vi "Main_Rover_Control.vi"() -> ()   [LabVIEW 2022 SP3]
doc: "Rows start at (0,0). Positive field inputs. Run once, Send Path, wait Path ready, Start. Persistent command replies exclude heartbeat. No headland."
panel:
  in  "Seed spacing cm (10 or 20)":i32=10
  in  "Enable planting":bool=TRUE
  out "Graph layout error":errorcluster
  in  "Orientation":enum16{"Run Along Length", "Run Along Width"}(ring)
  out "XY Graph":cluster{dbl[], dbl[]}(graph)={[0.0, 0.0, 2.0, 2.0, 4.0, 4.0, 6.0, 6.0], [0.0, 8.0, 8.0, 0.0, 0.0, 8.0, 8.0, 0.0]}
  in  "Row Spacing":dbl=2.0
  in  "Field Length":dbl=8.0
  in  "Field Width":dbl=6.0
  out "Field inputs valid":bool
  out "Connection error":errorcluster
  out "Expected acknowledgement":string
  out "Run status":string="Stopped"
  out "Last rover error":string
  out "Connected":bool
  out "Calibration valid":bool
  out "Running estimate":bool
  out "Path ready":bool
  out "Current command":string
  out "Last received line":string
  in  "Disconnect":bool
  in  "Reset E-stop":bool
  in  "E-STOP":bool
  in  "STOP":bool
  in  "Start":bool
  in  "Send Path":bool
  out "Path points":i32
  out "Greeting":string
  in  "Initial heading degrees":dbl=90.0
  in  "Right 90 ms - calibrate":dbl=925.0
  in  "Left 90 ms - calibrate":dbl=925.0
  in  "Forward ms per cm":dbl=40.0
  in  "TCP port":u16=5000
  in  "ESP32 address":string="192.168.4.1"
  # "ROVER PATH CONTROL"
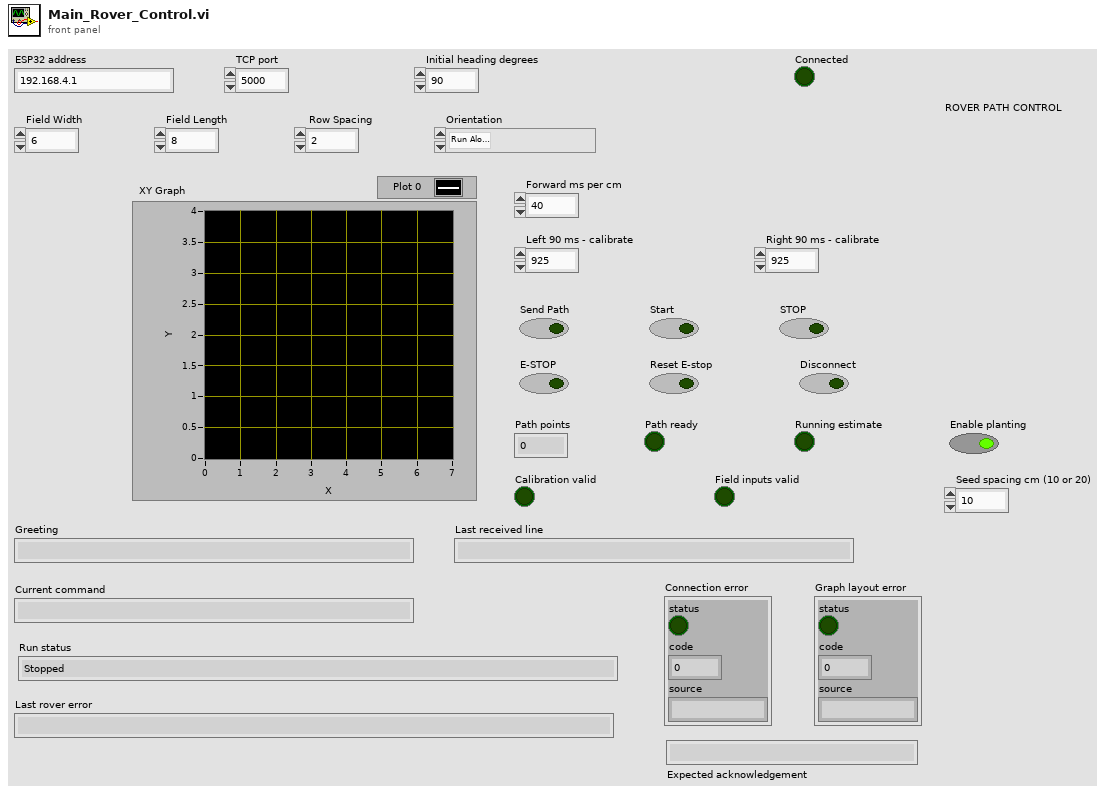
[diagram p1: front panel]
diagram:
  w97 = cluster{"Width":u32, "Height":u32} {"Width"=250, "Height"=250}  # Plot size
  w92 = 2.0  # x
  w88 = 3.0  # Safe s
  w86 = 6.0  # Safe l
  w84 = 5.0  # Safe w
  w83 = errorcluster {"status"=FALSE, "code"=0, "source"=""}  # Input error template
  w76 = 100  # Final timeout
  w75 = "STOP\r\n"  # Final STOP
  w70 = ""  # lastline initial
  w69 = ""  # wanted initial
  w68 = ""  # buffer initial
  w67 = 0  # oldreset initial
  w66 = 0  # oldestop initial
  w65 = 0  # oldstop initial
  w64 = 0  # oldstart initial
  w63 = 0  # oldsend initial
  w62 = 0  # lastreceive initial
  w61 = 0  # lastping initial
  w60 = 0  # running initial
  w59 = 0  # ready initial
  w58 = 0  # deadline initial
  w57 = 0  # pending initial
  w56 = -1  # position initial
  w51 = "HELLO,ROVER,2,CM_PER_UNIT=10\r\n"  # Expected greeting
  w47 = 30  # Greeting bytes
  w44 = 3000  # Connect timeout
  w41 = 3  # Decimals
  w40 = "START,"  # Start prefix
  w30 = "OK,CAL"  # Calibration acknowledgement
  w26 = 3  # Decimals
  w25 = ","  # Comma
  w23 = 3  # Decimals
  w22 = ","  # Comma
  w20 = 3  # Decimals
  w19 = "CAL,"  # CAL
  n1 = property on="XY Graph" class="XYGraph (strict)"("Plot Area:Size"=w97) -> (error out=→"Graph layout error":errorcluster)  [unwired: 2 in, 1 out]
  n2 = Number To Fractional String(number="Forward ms per cm", precision (6)=w20) -> (F-format string=w21:string)  [unwired: 2 out]
  n3 = Number To Fractional String(number="Left 90 ms - calibrate", precision (6)=w23) -> (F-format string=w24:string)  [unwired: 2 out]
  n4 = Number To Fractional String(number="Right 90 ms - calibrate", precision (6)=w26) -> (F-format string=w27:string)  [unwired: 2 out]
  n5 = Build Array(w30) -> (w31:string[])
  n6 = Number To Fractional String(number="Initial heading degrees", precision (6)=w41) -> (F-format string=w42:string)  [unwired: 2 out]
  n7 = TCP Open Connection(address="ESP32 address", remote port or service name="TCP port", timeout ms (60000)=w44) -> (connection ID=w45:refnum<k5>, error out=w46:errorcluster)  [unwired: 2 in]
  n8 = To Long Integer(number="Orientation") -> (32bit integer=w80:i32)
  n9 = Select(t="PLANT,1,", s="Enable planting", f="PLANT,0,") -> (s? t:f=w102:string)
  n10 = Number To Decimal String(number="Seed spacing cm (10 or 20)") -> (decimal integer string=w103:string)  [unwired: 1 in]
  n11 = Build Array("OK,PLANT") -> (w35:string[])
  n12 = Concatenate Strings(w19, w21, w22, w24, w25, w27) -> (w28:string)
  n13 = Concatenate Strings(w40, w42) -> (w43:string)
  n14 = TCP Read(connection ID=w45, bytes to read=w47, error in (no error)=w46, 9:w44) -> (connection ID out=w48:refnum<k5>, data out=w49:string, error out=w50:errorcluster)  [unwired: 1 in]
  "Greeting" <- w49
  "Connection error" <- w50
  n15 = formula code="int32 ok;float64 cross;ok=(w>0 && w<=1000 && l>0 && l<=1000 && s>0 && s<=1000 && (o==0 || o==1));if(ok){cross=w;if(o==1){cross=l;}ok=(cross/s<=127);}"("w"="Field Width", "l"="Field Length", "s"="Row Spacing", "o"=w80) -> ("ok"=w78:i32)
  n16 = Concatenate Strings(w102, w103) -> (w104:string)
  n17 = Build Array(w28) -> (w29:string[])
  n18 = Equal?(x=w49, y=w51) -> (x = y?=w52:bool)
  n19 = Unbundle By Name(w50) -> ("status"=w55:bool)
  n20 = Not Equal To 0?(x=w78) -> (x != 0?=w81:bool)
  "Field inputs valid" <- w81
  n21 = Build Array(w104) -> (w33:string[])
  n22 = Not(x=w81) -> (.not. x?=w82:bool)
  n23 = Select(t="Field Width", s=w81, f=w84) -> (s? t:f=w85:dbl)
  n24 = Select(t="Field Length", s=w81, f=w86) -> (s? t:f=w87:dbl)
  n25 = Select(t="Row Spacing", s=w81, f=w88) -> (s? t:f=w89:dbl)
  n26 = Bundle By Name(cluster=w83, "status"=w82) -> (w54:errorcluster)
  n27 = call "Generate_Rows.vi"("Orientation"="Orientation", "Row Spacing"=w89, "Field Length"=w87, "Field Width"=w85) -> ("Waypoints"=w93:cluster{"X":dbl, "Y":dbl, "Seed":bool}[][])  [unwired: 11 in]
  n28 = Unbundle By Name(w54) -> ("status"=w53:bool)
  n29 = Array Size(array=w93) -> (size(s)=w94:i32[])
  n30 = Index Array(array=w94) -> (element=w95:i32)  [unwired: 1 in]
  n31 = Multiply(x=w92, y=w95) -> (x*y=w96:dbl)
  n32 = for {
    N: w96 -> [_]
    tunnel: w93 -> [w111]
    tunnel: [w113] -> w11 mode=indexing
    tunnel: [w112] -> w10 mode=indexing
    tunnel: [w114] -> w12 mode=indexing
    i -> [w106]
    w107 = 2  # y
    n33 = Quotient & Remainder(x=w106, y=w107) -> (x-y*floor(x/y)=w109:i32, floor(x/y)=w108:i32)
    n34 = Index Array(array=w111, index (row)=w108, index (col)=w109) -> (element=w110:cluster{"X":dbl, "Y":dbl, "Seed":bool})
    n35 = Unbundle By Name(w110) -> ("X"=w112:dbl, "Y"=w113:dbl, "Seed"=w114:bool)
  }
  n36 = call "Rover_Planting_Commands.vi"("X"=w10, "Y"=w11, "Seeds"=w12) -> ("Commands"=w7:string[], "Expected"=w8:string[], "Count"=w9:i32)  [unwired: 10 in]
  "Path points" <- w9
  n37 = Array Size(array=w11) -> (size(s)=w13:i32)
  n38 = Bundle(w10, w11) -> (→"XY Graph":cluster{dbl[], dbl[]})  [unwired: 1 in]
  n39 = formula code="int32 ok,i;ok=(n>=2 && n<=256 && n==ny);if(ok){for(i=0;i<n;i++){if(!(x[i]>=-0.000001 && x[i]<=w+0.000001 && y[i]>=-0.000001 && y[i]<=l+0.000001)){ok=0;}}}"("n"=w9, "ny"=w13, "x"=w10, "y"=w11, "w"="Field Width", "l"="Field Length") -> ("ok"=w14:i32)
  n40 = formula code="int32 valid; valid=((spacing==10 || spacing==20) && n>=2 && n<=256 && n==ny && ms>=1 && ms<=1000 && l>=1 && l<=10000 && r>=1 && r<=10000 && h>=-180 && h<=180);"("n"=w9, "ny"=w13, "ms"="Forward ms per cm", "l"="Left 90 ms - calibrate", "r"="Right 90 ms - calibrate", "h"="Initial heading degrees", "spacing"="Seed spacing cm (10 or 20)") -> ("valid"=w17:i32)
  n41 = Build Array (concatenate)(w29, w7, w33) -> (w32:string[])
  n42 = Build Array (concatenate)(w31, w8, w35) -> (w34:string[])
  n43 = Not Equal To 0?(x=w17) -> (x != 0?=w36:bool)
  n44 = Select(t=w32, s=w36, f=w7) -> (s? t:f=w37:string[])
  n45 = Select(t=w34, s=w36, f=w8) -> (s? t:f=w38:string[])
  n46 = Array Size(array=w37) -> (size(s)=w39:i32)
  n47 = while {
    shift-right: [w129] -> _
    shift-left: w56 -> [w128]
    shift-right: [w131] -> _
    shift-left: w57 -> [w130]
    shift-right: [w133] -> _
    shift-left: w58 -> [w132]
    shift-right: [w135] -> _
    shift-left: w59 -> [w134]
    shift-right: [w137] -> _
    shift-left: w60 -> [w136]
    shift-right: [w139] -> _
    shift-left: w61 -> [w138]
    shift-right: [w141] -> _
    shift-left: w62 -> [w140]
    shift-right: [w143] -> _
    shift-left: w63 -> [w142]
    shift-right: [w145] -> _
    shift-left: w64 -> [w144]
    shift-right: [w147] -> _
    shift-left: w65 -> [w146]
    shift-right: [w149] -> _
    shift-left: w66 -> [w148]
    shift-right: [w151] -> _
    shift-left: w67 -> [w150]
    shift-right: [w153] -> _
    shift-left: w68 -> [w152]
    shift-right: [w155] -> _
    shift-left: w69 -> [w154]
    shift-right: [w229] -> _
    shift-left: w70 -> [w228]
    shift-right: [w232] -> _
    shift-left: "" -> [w239]
    shift-right: [w244] -> _
    shift-left: "" -> [w243]
    shift-right: [w246] -> _
    shift-left: 0 -> [w201]
    tunnel: w48 -> [w116]
    tunnel: w43 -> [w122]
    tunnel: w52 -> [w123]
    tunnel: w55 -> [w124]
    tunnel: w53 -> [w125]
    tunnel: w17 -> [w120]
    tunnel: w14 -> [w121]
    tunnel: w37 -> [w117]
    tunnel: w38 -> [w118]
    tunnel: w39 -> [w119]
    tunnel: [w222] -> w71
    tunnel: [w223] -> _
    i -> [w115]
    stop <- w226 stop-if-true
    w227 = u32 10  # UI polling delay
    w221 = 100  # Write timeout
    w219 = ""  # Empty write
    w216 = "\r\n"  # Line ending
    w212 = "OK,RESET"  # Reset ack
    w211 = "ESTOPPED"  # Estop ack
    w210 = "STOPPED"  # Stop ack
    w209 = "OK,START"  # Start ack
    w208 = "RESET"  # Reset command
    w207 = "ESTOP"  # Emergency stop
    w206 = "STOP"  # Stop command
    w205 = "PING"  # Heartbeat
    w204 = ""  # No command
    w190 = "ERR,"  # Error prefix
    w188 = 4  # Prefix length
    w185 = "DONE"  # Done
    w177 = "\r\n"  # CRLF
    w171 = u16 3  # Immediate mode
    w170 = 10  # Read timeout
    w169 = 1024  # Read chunk
    w127 = 1  # One
    w126 = 0  # Zero
    n48 = Tick Count (ms)() -> (millisecond timer value=w168:u32)
    n49 = Select(t=w127, s="Send Path", f=w126) -> (s? t:f=w157:i32)
    n50 = Select(t=w127, s="Start", f=w126) -> (s? t:f=w159:i32)
    n51 = Select(t=w127, s="STOP", f=w126) -> (s? t:f=w161:i32)
    n52 = Select(t=w127, s="E-STOP", f=w126) -> (s? t:f=w163:i32)
    n53 = Select(t=w127, s="Reset E-stop", f=w126) -> (s? t:f=w165:i32)
    n54 = Select(t=w127, s="Disconnect", f=w126) -> (s? t:f=w167:i32)
    n55 = Wait (ms)(milliseconds to wait=w227) -> ()  [unwired: 1 out]
    n56 = Build Array("Stopped", "Connected - click Send Path", "Uploading path - please wait", "Path ready - click Start", "Start sent - waiting / running", "Path completed", "Stopped - upload again to restart", "Emergency stop - Reset then upload", "Reset sent - upload path", "Start blocked - Send Path first", "Invalid field or path settings", "Invalid calibration, heading or seed spacing", "Rover rejected command - see Last rover error", "Command acknowledgement timed out", "Connection lost - no heartbeat reply", "Disconnected", "Upload blocked - rover is running", "Command pending - wait before retry", "TCP read failed - reconnect then Run", "TCP write failed - reconnect then Run", "Invalid or oversized incoming message", "Firmware greeting mismatch - protocol 2 required", "Connection failed - connect to Rover_AP then Run") -> (w271:string[])
    n57 = TCP Read(connection ID=w116, bytes to read=w169, 7:w171, 9:w170) -> (connection ID out=w172:refnum<k5>, data out=w173:string, error out=w174:errorcluster)  [unwired: 1 in]
    n58 = Select(t=w127, s=w123, f=w126) -> (s? t:f=w194:i32)
    n59 = Select(t=w127, s=w124, f=w126) -> (s? t:f=w195:i32)
    n60 = Select(t=w127, s=w125, f=w126) -> (s? t:f=w196:i32)
    n61 = Not Equal To 0?(x=w120) -> (x != 0?=→"Calibration valid":bool)
    n62 = Unbundle By Name(w174) -> ("code"=w175:i32)
    n63 = Concatenate Strings(w152, w173) -> (w176:string)
    n64 = Match Pattern(string=w176, regular expression=w177) -> (before substring=w178:string, after substring=w179:string, offset past match=w180:i32)  [unwired: 1 in, 1 out]
    n65 = String Length(string=w176) -> (length=w193:i32)
    n66 = formula code="int32 yes; yes=n>=0;"("n"=w180) -> ("yes"=w181:i32)
    n67 = Equal?(x=w178, y=w154) -> (x = y?=w183:bool)
    n68 = Equal?(x=w178, y=w185) -> (x = y?=w186:bool)
    n69 = String Subset(string=w178, length (rest)=w188) -> (substring=w189:string)  [unwired: 1 in]
    n70 = Not Equal?(x=w178, y="PONG") -> (x != y?=w238:bool)
    n71 = Not Equal To 0?(x=w181) -> (x != 0?=w182:bool)
    n72 = Select(t=w127, s=w183, f=w126) -> (s? t:f=w184:i32)
    n73 = Select(t=w127, s=w186, f=w126) -> (s? t:f=w187:i32)
    n74 = Equal?(x=w189, y=w190) -> (x = y?=w191:bool)
    n75 = Not Equal To 0?(x=w181) -> (x != 0?=w230:bool)
    n76 = Select(t=w179, s=w182, f=w176) -> (s? t:f=w153:string)
    n77 = Select(t=w127, s=w191, f=w126) -> (s? t:f=w192:i32)
    n78 = And(x=w230, y=w238) -> (x .and. y?=w231:bool)
    n79 = And(x=w230, y=w191) -> (x .and. y?=w245:bool)
    n80 = Select(t=w178, s=w231, f=w228) -> (s? t:f=w229:string)
    "Last received line" <- w229
    n81 = Select(t=w178, s=w245, f=w243) -> (s? t:f=w244:string)
    "Last rover error" <- w244
    n82 = formula code="int32 action,qi,quit,positionNext,pendingNext,deadlineNext,readyNext,runningNext,lastpingNext,lastreceiveNext,oldsendNext,oldstartNext,oldstopNext,oldestopNext,oldresetNext,diagnostic;\ndiagnostic=previousStatus;action=0; qi=position; quit=0; positionNext=position; pendingNext=pending; deadlineNext=deadline; readyNext=ready; runningNext=running; lastpingNext=lastping;lastreceiveNext=lastreceive;if(iteration==0 || complete){lastreceiveNext=now;}\noldsendNext=send; oldstartNext=start; oldstopNext=stop; oldestopNext=estop; oldresetNext=reset;\nif(complete && pending && ack){pendingNext=0; if(position>=0){positionNext=position+1;if(positionNext>=qlen){positionNext=-1;readyNext=1;}}}\nif(complete && done){runningNext=0;readyNext=0;diagnostic=5;}\nif(complete && remoteerr){positionNext=-1;pendingNext=0;readyNext=0;runningNext=0;action=4;diagnostic=12;}\nif((code!=0 && code!=56)||!good||ge||grapherr||blen>8192||(now-lastreceiveNext>1200)||(pending && now-deadline>1200)){quit=1;action=4;readyNext=0;runningNext=0;positionNext=-1;pendingNext=0;}\nif(!quit && send && !oldsend && pathvalid && valid && !runningNext && !pendingNext){positionNext=0;readyNext=0;}\nif(positionNext>=0 && !pendingNext){action=2;qi=positionNext;pendingNext=1;deadlineNext=now;}\nif(!quit && start && !oldstart && readyNext && valid && pathvalid && !pendingNext){action=3;readyNext=0;runningNext=1;pendingNext=1;deadlineNext=now;}\nif(reset && !oldreset){action=6;positionNext=-1;pendingNext=1;deadlineNext=now;readyNext=0;runningNext=0;}\nif(stop && !oldstop){action=4;positionNext=-1;pendingNext=1;deadlineNext=now;readyNext=0;runningNext=0;}\nif(estop && !oldestop){action=5;positionNext=-1;pendingNext=1;deadlineNext=now;readyNext=0;runningNext=0;}\nif(close){quit=1;action=4;}\nif(quit){action=4;runningNext=0;readyNext=0;positionNext=-1;}\nif(action==0 && now-lastping>200){action=1;}\nif(action!=0){lastpingNext=now;}\n\nif(iteration==0){diagnostic=1;}\nif(send && !oldsend){if(!pathvalid || grapherr){diagnostic=10;}else if(!valid){diagnostic=11;}else if(running){diagnostic=16;}else if(pending){diagnostic=17;}}\nif(start && !oldstart && !ready){diagnostic=9;}\nif(action==2){diagnostic=2;}\nif(readyNext){diagnostic=3;}\nif(action==3){diagnostic=4;}\nif(stop && !oldstop){diagnostic=6;}\nif(estop && !oldestop){diagnostic=7;}\nif(reset && !oldreset){diagnostic=8;}\nif(complete && remoteerr){diagnostic=12;}\nif(close){diagnostic=15;}\nif(pending && now-deadline>1200){diagnostic=13;}\nif(now-lastreceiveNext>1200){diagnostic=14;}\nif(blen>8192){diagnostic=20;}\nif(code!=0 && code!=56){diagnostic=18;}\nif(!good){diagnostic=21;}\nif(ge){diagnostic=22;}\nif(grapherr){diagnostic=10;}"("position"=w128, "pending"=w130, "deadline"=w132, "ready"=w134, "running"=w136, "lastping"=w138, "lastreceive"=w140, "oldsend"=w142, "oldstart"=w144, "oldstop"=w146, "oldestop"=w148, "oldreset"=w150, "send"=w157, "start"=w159, "stop"=w161, "estop"=w163, "reset"=w165, "close"=w167, "now"=w168, "ack"=w184, "done"=w187, "remoteerr"=w192, "complete"=w181, "code"=w175, "qlen"=w119, "valid"=w120, "pathvalid"=w121, "good"=w194, "ge"=w195, "grapherr"=w196, "blen"=w193, "iteration"=w115, "previousStatus"=w201) -> ("action"=w197:i32, "qi"=w198:i32, "quit"=w199:i32, "positionNext"=w129:i32, "pendingNext"=w131:i32, "deadlineNext"=w133:i32, "readyNext"=w135:i32, "runningNext"=w137:i32, "lastpingNext"=w139:i32, "lastreceiveNext"=w141:i32, "oldsendNext"=w143:i32, "oldstartNext"=w145:i32, "oldstopNext"=w147:i32, "oldestopNext"=w149:i32, "oldresetNext"=w151:i32, "diagnostic"=w200:i32)
    n83 = Index Array(array=w117, index=w198) -> (element=w202:string)
    n84 = Index Array(array=w118, index=w198) -> (element=w203:string)
    n85 = Not Equal To 0?(x=w197) -> (x != 0?=w218:bool)
    n86 = Not Equal To 0?(x=w199) -> (x != 0?=w225:bool)
    n87 = Not Equal To 0?(x=w135) -> (x != 0?=→"Path ready":bool)
    n88 = Not Equal To 0?(x=w137) -> (x != 0?=w234:bool)
    n89 = formula code="int32 yes;yes=a>=2;"("a"=w197) -> ("yes"=w240:i32)
    n90 = Not Equal To 0?(x=w199) -> ()  [unwired: 1 out]
    n91 = Build Array(w204, w205, w202, w122, w206, w207, w208) -> (w213:string[])
    n92 = Build Array(w154, w154, w203, w209, w210, w211, w212) -> (w214:string[])
    n93 = Not Equal To 0?(x=w240) -> (x != 0?=w241:bool)
    n94 = Index Array(array=w213, index=w197) -> (element=w215:string)
    n95 = Index Array(array=w214, index=w197) -> (element=w155:string)
    n96 = Concatenate Strings(w215, w216) -> (w217:string)
    n97 = Select(t=w215, s=w241, f=w239) -> (s? t:f=w232:string)
    "Current command" <- w232
    n98 = Select(t=w217, s=w218, f=w219) -> (s? t:f=w220:string)
    n99 = TCP Write(connection ID=w172, data in=w220, 9:w221) -> (connection ID out=w222:refnum<k5>, error out=w223:errorcluster)  [unwired: 1 in, 1 out]
    n100 = Unbundle By Name(w223) -> ("status"=w224:bool)
    n101 = Or(x=w225, y=w224) -> (x .or. y?=w226:bool)
    n102 = Select(t=19, s=w224, f=w200) -> (s? t:f=w246:i32)
    n103 = Not(x=w226) -> (.not. x?=→"Connected":bool)
    n104 = Index Array(array=w271, index=w246) -> (element=→"Run status":string)
    n105 = Not(x=w226) -> (.not. x?=w273:bool)
    n106 = And(x=w234, y=w273) -> (x .and. y?=→"Running estimate":bool)
    "Expected acknowledgement" <- w154
  }
  n107 = TCP Write(connection ID=w71, data in=w75, 9:w76) -> (connection ID out=w77:refnum<k5>)  [unwired: 1 in, 2 out]
  n108 = TCP Close Connection(connection ID=w77) -> ()  [unwired: 2 in, 2 out]
